vi "GO alertes Compteurs.vi"(5 "Numéro":u8) -> ()   [LabVIEW 2022 SP3]
uses:
  Enum/Enum s1.ctl
  Variables globales/Variable glob alertes Compteurs.vi
  Variables globales/Variable glob mails.vi
  Variables globales/Variable globale compteurs.vi
  Variables globales/Variable glob generale.vi
panel:
  out "défaut max compt":bool
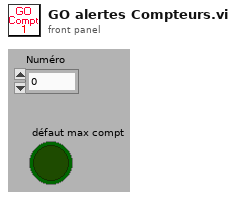
[diagram p1: front panel]
types:
  T1 = typedef "Enum s1.ctl" = enum16{"Alerte vide", "Alerte temperature min-max", "Alerte temperature ecart", "Alerte Keller", "Alerte compteur", "Alerte régulateurs"}
  T2 = cluster{"Alerte":bool, "valeur alerte":dbl, "Défaut":bool, "Indices à controler":i16[], "N°":u16}[]
  T3 = cluster{"Alerte":bool, "valeur alerte":dbl, "Défaut":bool, "Indices à controler":i16[], "N°":u16}
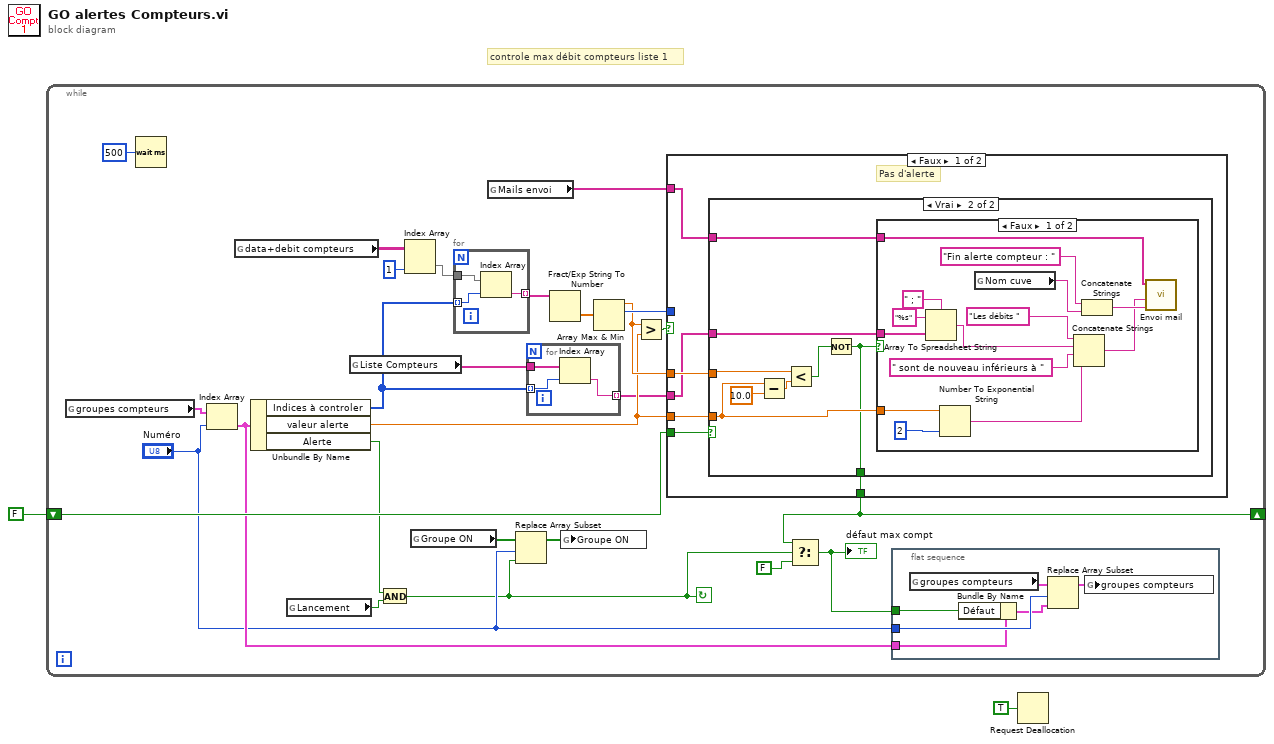
[diagram p0: block diagram]
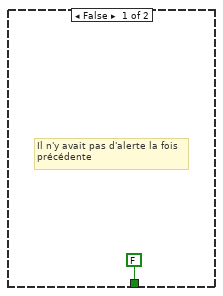
[diagram p2: hidden frame]
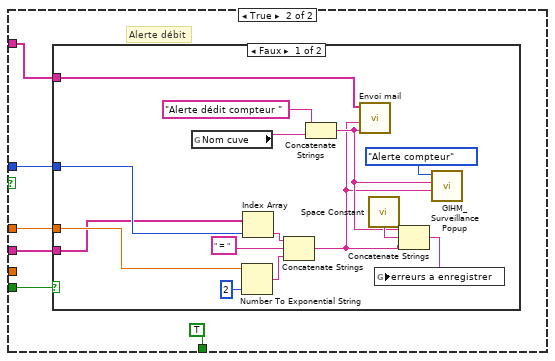
[diagram p4: hidden frame]
diagram:
  # "controle max débit compteurs liste 1"
  n1 = while {
    shift-right: [w12] -> _
    shift-left: FALSE -> [w26]
    stop <- w4 continue-if-true
    n2 = global read "Variable glob alertes Compteurs.vi" "groupes compteurs"() -> (w16:T2)
    n3 = Wait (ms)(milliseconds to wait=u32 500 ("attente (ms)")) -> ()  [unwired: 1 out]
    n4 = Index Array(array=w16, index="Numéro") -> (element=w14:T3)
    n5 = global read "Variable globale compteurs.vi" "data+debit compteurs"() -> (w19:string[][])
    n6 = Unbundle By Name(w14) -> ("Indices à controler"=w10:i16[], "valeur alerte"=w15:dbl, "Alerte"=w8:bool)
    n7 = global read "Variable glob generale.vi" "Lancement"() -> (w21:bool)
    n8 = global read "Variable glob alertes Compteurs.vi" "Liste Compteurs"() -> (w11:string[])
    n9 = And(x=w8, y=w21) -> (x .and. y?=w4:bool)
    n10 = Index Array(array=w19, index (col)=1 ("indice désactivé (col)")) -> (element=w17:string[])  [unwired: 1 in]
    n11 = global read "Variable glob alertes Compteurs.vi" "Groupe ON"() -> (w6:bool[])
    n12 = for {
      tunnel: w17 -> [w89]
      tunnel: w10 -> [w90] mode=indexing
      tunnel: [w88] -> w28 mode=indexing
      n13 = Index Array(array=w89, index=w90) -> (element=w88:string)
    }
    n14 = global read "Variable glob mails.vi" "Mails envoi"() -> (w7:string[])
    n15 = Replace Array Subset(array=w6, new element=w4, index="Numéro") -> (w3:bool[])
    n16 = for {
      tunnel: w10 -> [w30] mode=indexing
      tunnel: w11 -> [w31]
      tunnel: [w29] -> w9 mode=indexing
      n17 = Index Array(array=w31, index=w30) -> (element=w29:string)
    }
    n18 = Fract/Exp String To Number(string=w28) -> (number=w22:dbl[])  [unwired: 3 in, 1 out]
    n19 = global write "Variable glob alertes Compteurs.vi" "Groupe ON"(w3) -> ()
    n20 = Array Max & Min(array=w22) -> (max value=w24:dbl, max index (indices)=w25:i32)  [unwired: 2 out]
    n21 = Greater?(x=w24, y=w15) -> (0:w23:bool)
    n22 = case shown="Faux" w23 {
      tunnel: w26 -> [w42 w72]
      tunnel: w25 -> [_ w71]
      tunnel: w24 -> [w40 w70]
      tunnel: w15 -> [w43 _]
      tunnel: w7 -> [w41 w69]
      tunnel: [w39 TRUE] -> w12
      tunnel: w9 -> [w38 w67]
      frame False {
        # "Pas d'alerte"
        n23 = case shown="Vrai" w42 {
          tunnel: w43 -> [_ w47]
          tunnel: w41 -> [_ w52]
          tunnel: w40 -> [_ w51]
          tunnel: [FALSE w46] -> w39
          tunnel: w38 -> [_ w45]
          frame False {
            # "Il n'y avait pas d'alerte la fois\nprécédente"
          }
          frame True {
            n24 = Subtract(x=w47, y=10.0 ("x")) -> (x-y=w50:dbl)
            n25 = Less?(x=w51, y=w50) -> (x < y?=w49:bool)
            n26 = Not(x=w49) -> (.not. x?=w46:bool)
            n27 = case shown="Faux" w46 {
              tunnel: w47 -> [w66 _]
              tunnel: w52 -> [w63 _]
              tunnel: w45 -> [w60 _]
              frame False {
                n28 = Array To Spreadsheet String(delimiter (Tab)=" ; " ("séparateur (Tabulation)"), array=w60, 3:"%s" ("chaîne de format")) -> (spreadsheet string=w56:string)
                n29 = Number To Exponential String(number=w66, precision (6)=i16 2 ("précision (6)")) -> (E-format string=w54:string)  [unwired: 2 in]
                n30 = global read "Variable glob generale.vi" "Nom cuve"() -> (w61:string)
                n31 = Concatenate Strings("Les débits ", w56, " sont de nouveau inférieurs à ", w54) -> (w53:string)
                n32 = Concatenate Strings("Fin alerte compteur : " ("subject ([No Subject])"), w61) -> (w62:string)
                n33 = call "Envoi mail.vi"("Objet"=w62, "Message"=w53, "Mail liste"=w63) -> ()  [unwired: 3 in]
              }
              frame True {
              }
            }
          }
        }
      }
      frame True {
        # "Alerte débit"
        n34 = case shown="Faux" w72 {
          tunnel: w71 -> [w84 _]
          tunnel: w70 -> [w83 _]
          tunnel: w69 -> [w80 _]
          tunnel: w67 -> [w78 _]
          frame False {
            n35 = global read "Variable glob generale.vi" "Nom cuve"() -> (w79:string)
            n36 = Number To Exponential String(number=w83, precision (6)=i16 2 ("précision (6)")) -> (E-format string=w86:string)  [unwired: 2 in]
            n37 = Index Array(array=w78, index=w84) -> (element=w85:string)
            n38 = Concatenate Strings(w85, " = " ("chaîne"), w86) -> (w74:string)
            n39 = Concatenate Strings("Alerte dédit compteur " ("subject ([No Subject])"), w79) -> (w75:string)
            n40 = call "Envoi mail.vi"("Objet"=w75, "Message"=w74, "Mail liste"=w80) -> ()  [unwired: 3 in]
            n41 = call <vilib>:"Space Constant.vi"() -> ("String"=w76:string)
            n42 = Concatenate Strings(w75, w76, w74) -> (w77:string)
            n43 = global write "Variable glob generale.vi" "erreurs a enregistrer"(w77) -> ()
            n44 = call "GIHM_Surveillance Popup.vi"("Message"=w74, "Problème observé"=w75, "Type problème"=Enum_s1."Alerte compteur") -> ()  [unwired: 2 in, 1 out]
          }
          frame True {
            # "L'alerte était déjà présente"
          }
        }
      }
    }
    n45 = Select(t=w12, s=w4, f=FALSE ("cas faux")) -> (s? t:f=w13:bool)
    "défaut max compt" <- w13
    n46 = flat-sequence {
      tunnel: "Numéro" -> [w36]
      tunnel: w14 -> [w35]
      tunnel: w13 -> [w34]
      frame #0 {
        n47 = global read "Variable glob alertes Compteurs.vi" "groupes compteurs"() -> (w37:T2)
        n48 = Bundle By Name(cluster=w35, "Défaut"=w34) -> (w33:T3)
        n49 = Replace Array Subset(array=w37, new element=w33, index=w36) -> (w32:T2)
        n50 = global write "Variable glob alertes Compteurs.vi" "groupes compteurs"(w32) -> ()
      }
    }
  }
  n51 = Request Deallocation(TRUE ("flag")) -> ()
